vi "hid_Write.vi"() -> ()   [LabVIEW 2017]
uses:
  <userlib>/HID_ARZ/HID_ARZ.lvlib
panel:
  out "resulting string":string
  out "Coneccion":bool
  in  "LED2":bool
  in  "LED1":bool
  in  "M2":dbl(knob) scale=0.0..100.0
  in  "M1":dbl(knob) scale=0.0..100.0
  in  "stop":bool
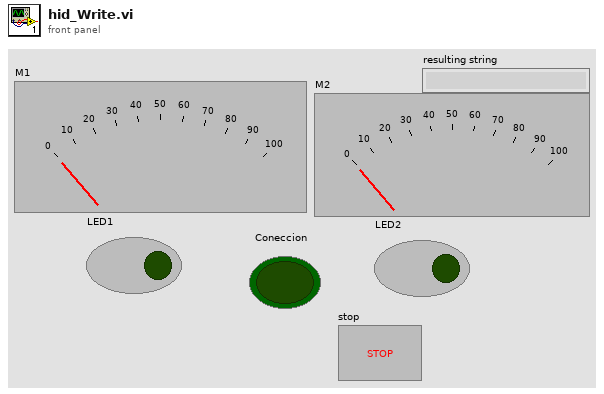
[diagram p1: front panel]
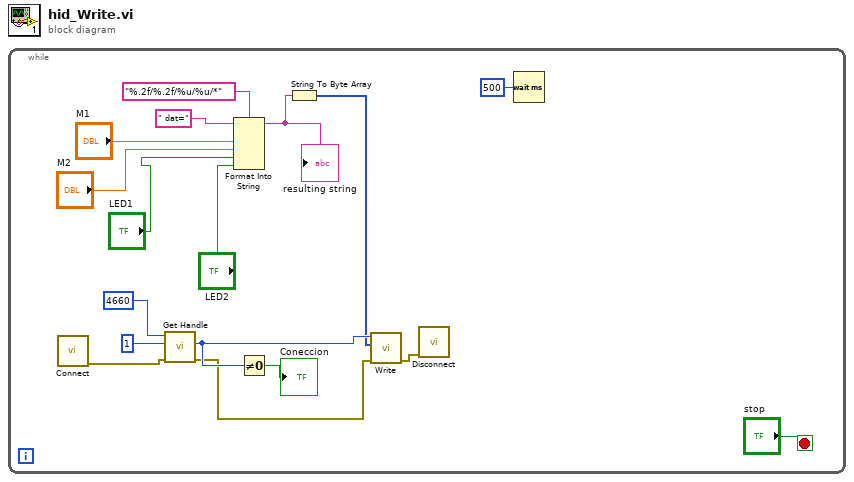
[diagram p0: block diagram]
diagram:
  n1 = while {
    stop <- "stop" stop-if-true
    n2 = call <userlib>:"Connect.vi"() -> ("error out"=w11:errorcluster)  [unwired: 9 in, 2 out]
    n3 = call <userlib>:"Get Handle.vi"("error in (no error)"=w11, "PID"=u32 1, "VID"=u32 4660) -> ("error out"=w7:errorcluster, "HANDLE"=w9:u32)  [unwired: 7 in]
    n4 = Format Into String(format string="%.2f/%.2f/%u/%u/*", initial string=" dat=", "M1", "M2", "LED1", "LED2") -> (resulting string=w1:string)  [unwired: 1 in, 1 out]
    "resulting string" <- w1
    n5 = Not Equal To 0?(x=w9) -> (x != 0?=→"Coneccion":bool)
    n6 = String To Byte Array(string=w1) -> (unsigned byte array=w8:u8[])
    n7 = call <userlib>:"Write.vi"("HANDLE"=w9, "DATOS"=w8, "error in (no error)"=w7) -> ("error out"=w6:errorcluster)  [unwired: 6 in, 1 out]
    n8 = call <userlib>:"Disconnect.vi"("error in (no error)"=w6) -> ()  [unwired: 10 in, 1 out]
    n9 = Wait (ms)(milliseconds to wait=u32 500) -> ()  [unwired: 1 out]
  }
